vi "test Get Owning Custom Device.vi"(8 "error in":errorcluster, 11 "TestCase in":refnum<class "Scripting.lvclass">) -> (0 "error out":errorcluster, 3 "TestCase out":refnum<class "Scripting.lvclass">)   [LabVIEW 2020, in "Scripting.lvclass"]
uses:
  Scripting.lvclass
  Shared/VS Channels Definition for Label.ctl
  Shared/VS Channel Definition for Parameter.ctl
  Shared/Parameter Definition.ctl
  <vilib>/NI/NI VeriStand Encoding and Decoding/Encoding.ctl
  Shared/Transfer Type.ctl
  Scripting.lvclass/Scripting.ctl
  Shared/Direction.ctl
  Shared/Transfer Speed.ctl
  <vilib>/addons/_JKI Toolkits/VI Tester/TestCase.llb/TestCase.lvclass
  Scripting/AIM/AIM ARINC 429 Scripting.lvlib
  <vilib>/NI/NI VeriStand Encoding and Decoding/Encoding and Decoding.lvlib
  C:/Program Files (x86)/National Instruments/LabVIEW 2020/vi.lib/addons/_JKI Toolkits/VI Tester/TestCase.llb/TestCase.lvclass
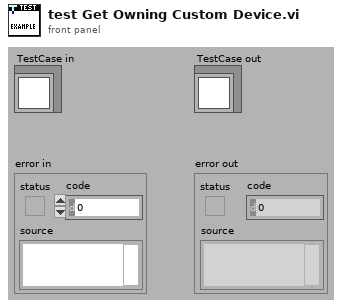
[diagram p1: front panel]
types:
  T1 = typedef "VS Channels Definition for Label.ctl" = cluster{"label (Dec)":u32, "parameters":T2[], "SDI value":u8, "SDI enabled":bool, "transfer type":T5, "create timestamp":bool, "transmit period":u32}
  T2 = typedef "VS Channel Definition for Parameter.ctl" = cluster{"name":string, "unit":string, "Parameter":T3}
  T3 = typedef "Parameter Definition.ctl" = cluster{"start index":i32, "size":i32, "encoding":T4, "signed":bool, "scale multiplier":dbl, "scale offset":dbl, "default value":dbl}
  T4 = typedef "Encoding and Decoding.lvlib/Encoding.ctl" = enum16{"BNR", "BCD", "Discrete"}
  T5 = typedef "Transfer Type.ctl" = enum16{"Scheduled", "Acyclic", "Block", "Strobe"}
  T6 = typedef "Transfer Speed.ctl" = enum16{"LO (12.5 kb/s)", "HI (100 kb/s)"}
  T7 = typedef "Direction.ctl" = enum16{"Rx", "Tx"}
  T8 = typedef "Custom Device API.lvlib/Custom Device Item Ref.ctl" = u64
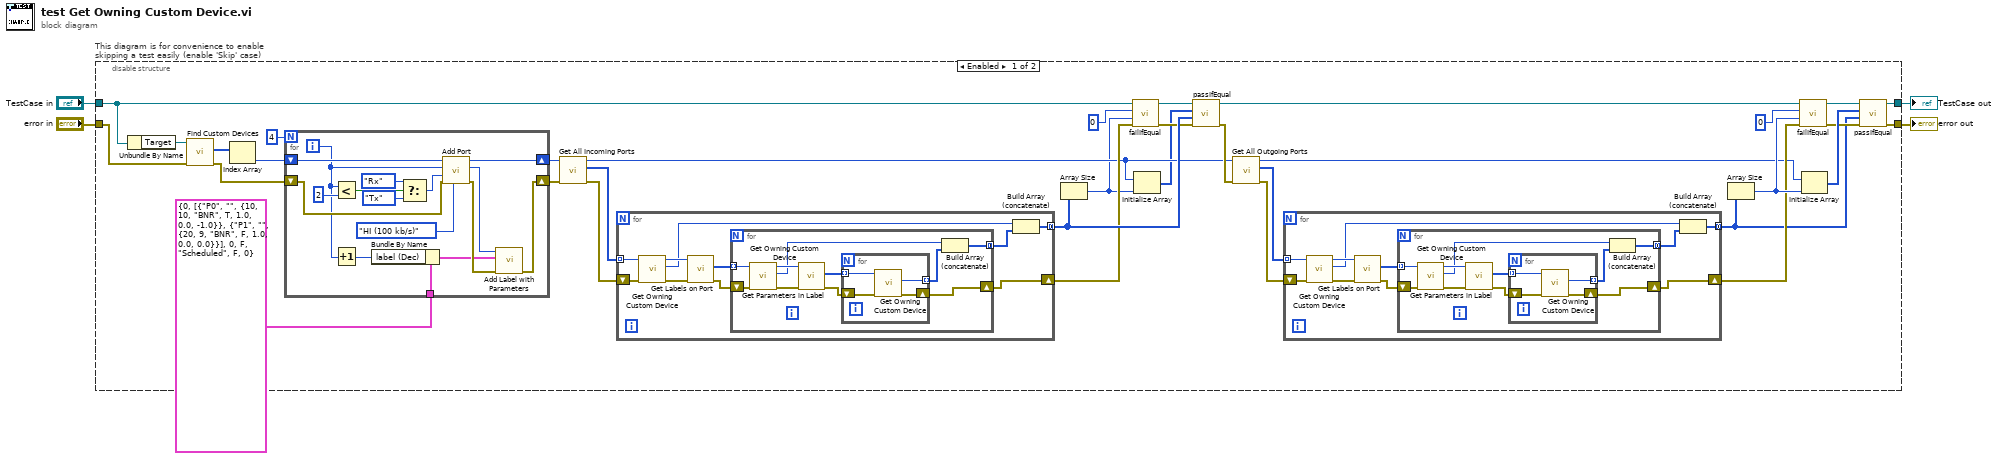
[diagram p0: block diagram]
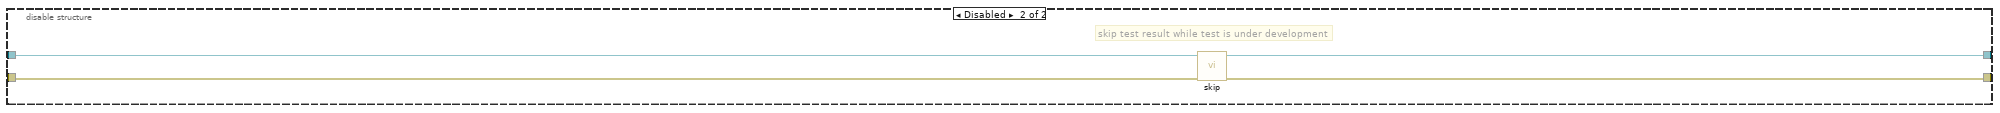
[diagram p2: hidden frame]
diagram:
  n1 = disable-structure "This diagram is for convenience to enable skipping a test easily (enable 'Skip' case)" shown="Enabled" {
    disable-tunnel: "TestCase in" -> [w30 w106]
    disable-tunnel: [w12 w104] -> w1
    disable-tunnel: [w13 w105] -> w3
    disable-tunnel: "error in" -> [w35 w103]
    frame Enabled {
      n2 = Unbundle By Name(w30) -> ("Target"=w38:refnum<k24>)
      n3 = call "Find Custom Devices.vi"("error in"=w35, "target"=w38) -> ("error out"=w7:errorcluster, "AIM ARINC 429 custom devices"=w11:T8[])  [unwired: 7 in, 1 out]
      n4 = Index Array(array=w11) -> (element=w10:T8)  [unwired: 1 in]
      n5 = for {
        N: 4 -> [_]
        shift-right: [w53] -> w9
        shift-left: w10 -> [w54]
        shift-right: [w40] -> w6
        shift-left: w7 -> [w47]
        tunnel: T1 {"label (Dec)"=0, "parameters"=[{"name"="P0", "unit"="", "Parameter"={"start index"=10, "size"=10, "encoding"=enum."BNR", "signed"=TRUE, "scale multiplier"=1.0, "scale offset"=0.0, "default value"=-1.0}}, {"name"="P1", "unit"="", "Parameter"={"start index"=20, "size"=9, "encoding"=enum."BNR", "signed"=FALSE, "scale multiplier"=1.0, "scale offset"=0.0, "default value"=0.0}}], "SDI value"=0, "SDI enabled"=FALSE, "transfer type"=enum."Scheduled", "create timestamp"=FALSE, "transmit period"=0} ("label") -> [w41]
        i -> [w44]
        n6 = Less?(x=w44, y=2) -> (x < y?=w51:bool)
        n7 = Increment(x=w44) -> (x+1=w43:i32)
        n8 = Bundle By Name(cluster=w41, "label (Dec)"=w43) -> (w42:T1)
        n9 = Select(t=Direction."Rx" ("direction"), s=w51, f=Direction."Tx" ("direction")) -> (s? t:f=w48:T7)
        n10 = call "Add Port.vi"("speed"=Transfer_Speed."HI (100 kb/s)", "error in"=w47, "direction"=w48, "port number"=w44, "custom device ref"=w54) -> ("error out"=w45:errorcluster, "port"=w46:T8, "custom device ref out"=w53:T8)  [unwired: 4 in]
        n11 = call "Add Label with Parameters.vi"("error in"=w45, "label"=w42, "port ref"=w46) -> ("error out"=w40:errorcluster)  [unwired: 7 in, 1 out]
      }
      n12 = call "Get All Incoming Ports.vi"("error in"=w6, "custom device ref"=w9) -> ("error out"=w37:errorcluster, "incoming ports"=w36:T8[], "custom device ref out"=w27:T8)  [unwired: 7 in]
      n13 = for {
        tunnel: w36 -> [w88] mode=indexing
        shift-right: [w82] -> w29
        shift-left: w37 -> [w87]
        tunnel: [w79] -> w33 mode=concatenating
        n14 = call "Get Owning Custom Device.vi"("error in"=w87, "item ref in"=w88) -> ("error out"=w85:errorcluster, "owning AIM ARINC-429 custom device"=w80:T8, "item ref out"=w86:T8)  [unwired: 7 in]
        n15 = call "Get Labels on Port.vi"("error in"=w85, "port ref"=w86) -> ("error out"=w83:errorcluster, "labels"=w84:T8[])  [unwired: 6 in, 2 out]
        n16 = for {
          tunnel: w84 -> [w98] mode=indexing
          shift-right: [w94] -> w82
          shift-left: w83 -> [w96]
          tunnel: [w89] -> w81 mode=concatenating
          n17 = call "Get Owning Custom Device.vi"("error in"=w96, "item ref in"=w98) -> ("error out"=w95:errorcluster, "owning AIM ARINC-429 custom device"=w91:T8, "item ref out"=w97:T8)  [unwired: 7 in]
          n18 = call "Get Parameters in Label.vi"("error in"=w95, "label ref"=w97) -> ("error out"=w92:errorcluster, "parameters"=w93:T8[])  [unwired: 6 in, 2 out]
          n19 = for {
            tunnel: w93 -> [w102] mode=indexing
            tunnel: [w101] -> w90 mode=indexing
            shift-right: [w99] -> w94
            shift-left: w92 -> [w100]
            n20 = call "Get Owning Custom Device.vi"("error in"=w100, "item ref in"=w102) -> ("error out"=w99:errorcluster, "owning AIM ARINC-429 custom device"=w101:T8)  [unwired: 7 in, 1 out]
          }
          n21 = Build Array (concatenate)(w91, w90) -> (w89:T8[])
        }
        n22 = Build Array (concatenate)(w80, w81) -> (w79:T8[])
      }
      n23 = Array Size(array=w33) -> (size(s)=w26:i32)
      n24 = call-dynamic "failIfEqual.vi"("error in (no error)"=w29, "y"=w26, "x"=0 ("size(s)"), "TestCase in"=w30) -> ("error out"=w28:errorcluster, "TestCase out"=w31:refnum<class "Scripting.lvclass">)  [unwired: 6 in]
      n25 = Initialize Array(w27, w26) -> (w25:T8[])
      n26 = call-dynamic "passIfEqual.vi"("error in (no error)"=w28, "y"=w33, "x"=w25, "TestCase in"=w31) -> ("error out"=w34:errorcluster, "TestCase out"=w15:refnum<class "Scripting.lvclass">)  [unwired: 6 in]
      n27 = call "Get All Outgoing Ports.vi"("error in"=w34, "custom device ref"=w27) -> ("error out"=w17:errorcluster, "outgoing ports"=w16:T8[], "custom device ref out"=w14:T8)  [unwired: 7 in]
      n28 = for {
        tunnel: w16 -> [w64] mode=indexing
        shift-right: [w58] -> w21
        shift-left: w17 -> [w63]
        tunnel: [w55] -> w18 mode=concatenating
        n29 = call "Get Owning Custom Device.vi"("error in"=w63, "item ref in"=w64) -> ("error out"=w61:errorcluster, "owning AIM ARINC-429 custom device"=w56:T8, "item ref out"=w62:T8)  [unwired: 7 in]
        n30 = call "Get Labels on Port.vi"("error in"=w61, "port ref"=w62) -> ("error out"=w59:errorcluster, "labels"=w60:T8[])  [unwired: 6 in, 2 out]
        n31 = for {
          tunnel: w60 -> [w74] mode=indexing
          shift-right: [w70] -> w58
          shift-left: w59 -> [w72]
          tunnel: [w65] -> w57 mode=concatenating
          n32 = call "Get Owning Custom Device.vi"("error in"=w72, "item ref in"=w74) -> ("error out"=w71:errorcluster, "owning AIM ARINC-429 custom device"=w67:T8, "item ref out"=w73:T8)  [unwired: 7 in]
          n33 = call "Get Parameters in Label.vi"("error in"=w71, "label ref"=w73) -> ("error out"=w68:errorcluster, "parameters"=w69:T8[])  [unwired: 6 in, 2 out]
          n34 = for {
            tunnel: w69 -> [w78] mode=indexing
            tunnel: [w77] -> w66 mode=indexing
            shift-right: [w75] -> w70
            shift-left: w68 -> [w76]
            n35 = call "Get Owning Custom Device.vi"("error in"=w76, "item ref in"=w78) -> ("error out"=w75:errorcluster, "owning AIM ARINC-429 custom device"=w77:T8)  [unwired: 7 in, 1 out]
          }
          n36 = Build Array (concatenate)(w67, w66) -> (w65:T8[])
        }
        n37 = Build Array (concatenate)(w56, w57) -> (w55:T8[])
      }
      n38 = Array Size(array=w18) -> (size(s)=w23:i32)
      n39 = call-dynamic "failIfEqual.vi"("error in (no error)"=w21, "y"=w23, "x"=0 ("size(s)"), "TestCase in"=w15) -> ("error out"=w22:errorcluster, "TestCase out"=w20:refnum<class "Scripting.lvclass">)  [unwired: 6 in]
      n40 = Initialize Array(w14, w23) -> (w24:T8[])
      n41 = call-dynamic "passIfEqual.vi"("error in (no error)"=w22, "y"=w18, "x"=w24, "TestCase in"=w20) -> ("error out"=w13:errorcluster, "TestCase out"=w12:refnum<class "Scripting.lvclass">)  [unwired: 6 in]
    }
    frame Disabled {
      # "skip test result while test is under development"
      n42 = call <vilib>:"skip.vi"("error in (no error)"=w103, "TestCase in"=w106) -> ("error out"=w105:errorcluster, "TestCase out"=w104:refnum<class "Scripting.lvclass">)  [unwired: 8 in]
    }
  }
  "error out" <- w3
  "TestCase out" <- w1
